vi "GetClassInfoDialog.vi"(0 "ClassWriterRefIn":refnum<class "ClassWriterNative.lvclass">, 1 "ClassItemRefIn":refnum<vi>, 5 "error in (no error)":errorcluster) -> (14 "ClassWriterRefOut":refnum<class "ClassWriterNative.lvclass">, 19 "error out":errorcluster)   [LabVIEW 2020, in "ClassWriterNative.lvclass"]
uses:
  <resource>/Framework/Providers/Open_GDS/ClassProviders/Provider_LvNativeClass/ClassWriterNative_class/ClassWriterNative.lvclass
  <resource>/Framework/Providers/Open_GDS/ClassProviders/Common/ScriptingFunctions/Scripting_ConnectorPanePatternType.ctl
  <resource>/Framework/Providers/Open_GDS/ClassProviders/Common/LvClass_class/GDSLvClass_PlugIn.ctl
  <resource>/Framework/Providers/Open_GDS/ClassProviders/Common/LvClass_class/GDSLvClass_PlugInTypes.ctl
  Instance           1 26Saved   GetClassInfoDialog .vi
  <resource>/Framework/Providers/Open_GDS/ClassProviders/Provider_LvNativeClass/ClassWriterNative_class/ClassWriterNative.lvclass/ClassWriterNative.ctl
panel:
  in  "Help":bool
  in  "_ShowContextHelp":bool
  in  "_SaveChanges":bool
  in  "_OK":bool
  out "ProductPicture":picture
  out "Connector Pane":T1 items=["4x4x4", "5x6x5", "6x8x6"]
  in  "_ClassPlugIns":T2(array[cluster]) caption="PlugIns / Design Patterns"
  in  "_EditPlugIn":bool
  out "_ClassDescription":string caption="Class description"
  out "_ClassTemplateVersion":string caption="Class Template Version"
  out "_ClassTemplateUsed":string caption="Class Template Used"
  out "_ClassProviderName":string caption="Class Provider Name"
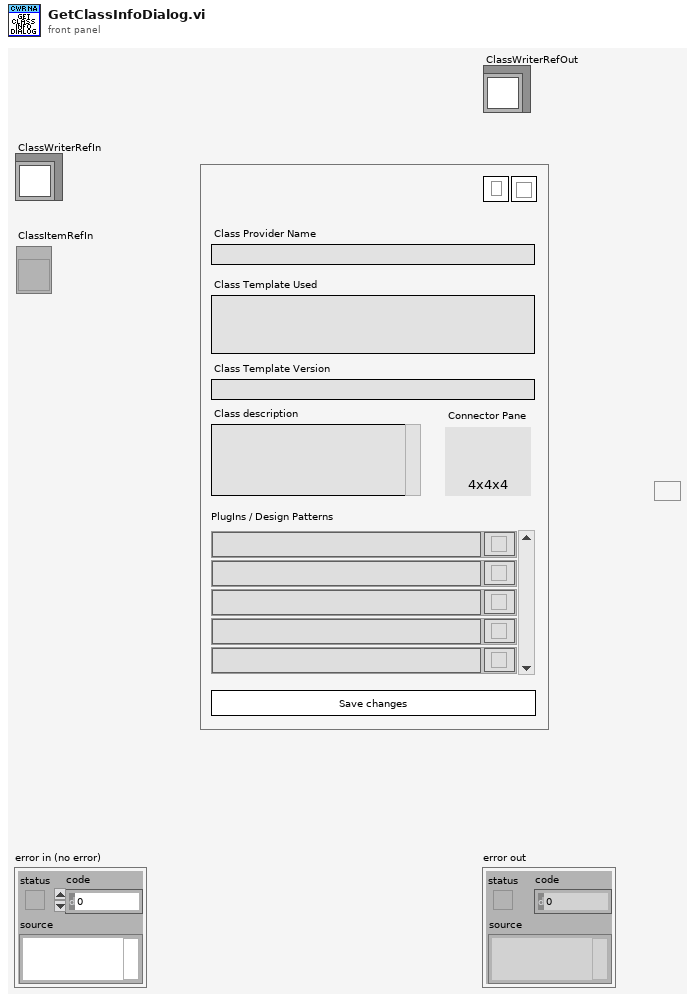
[diagram p1: front panel]
types:
  T1 = typedef "Scripting_ConnectorPanePatternType.ctl" = u16
  T2 = cluster{"_ClassPlugIn 2":string, "Remove":bool, "Block":bool}[]
  T3 = typedef "GDSLvClass_PlugIn.ctl" = cluster{"Type":T4, "ID":string, "Version":string, "Path":path, "Name":string, "Data":variant}
  T4 = typedef "GDSLvClass_PlugInTypes.ctl" = enum16{"DesignPattern", "MethodTypes"}
  T5 = cluster{"_ClassPlugIn 2":string, "_RemovePlugIn":bool, "Block":bool}
  T6 = typedef "GDSLvCLass_ClassSettingsType.ctl" = cluster{"ClassProviderName":string, "ClassTemplateUsed":string, "ClassTemplateVersion":string, "ClassDescription":string, "PlugIns":T3[], "ConnectorPanePattern":string}
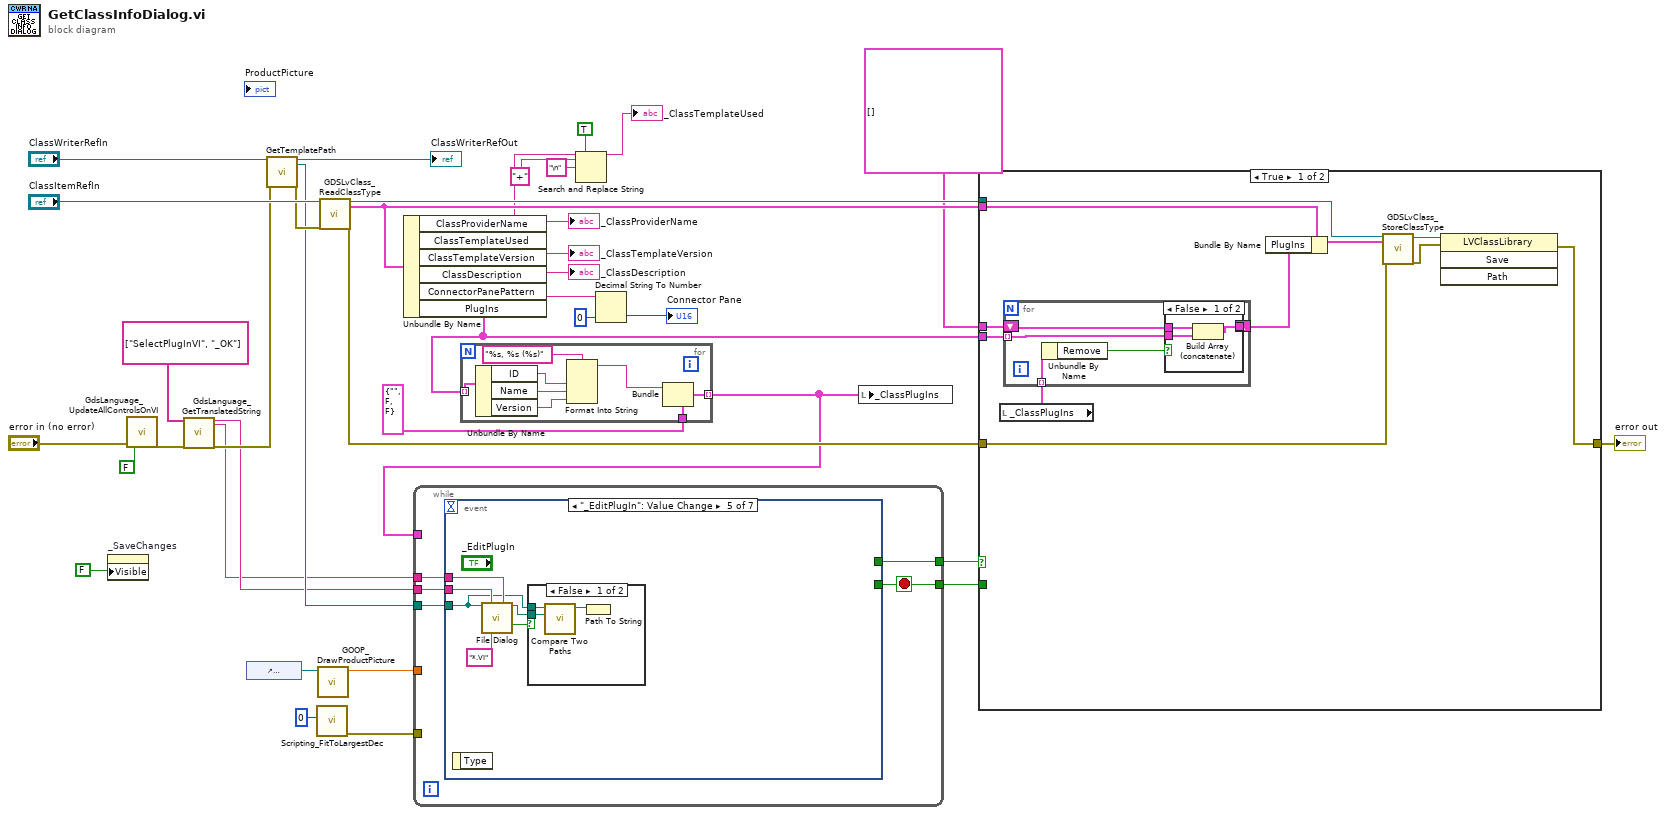
[diagram p0: block diagram]
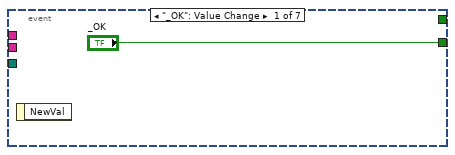
[diagram p4: hidden frame]
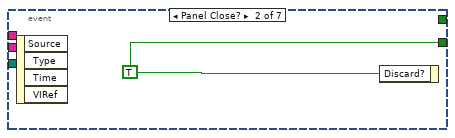
[diagram p5: hidden frame]
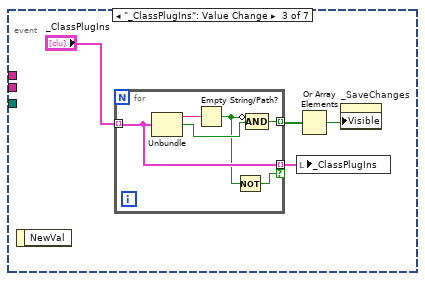
[diagram p6: hidden frame]
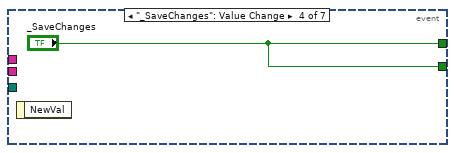
[diagram p7: hidden frame]
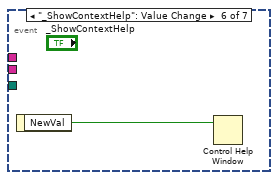
[diagram p9: hidden frame]
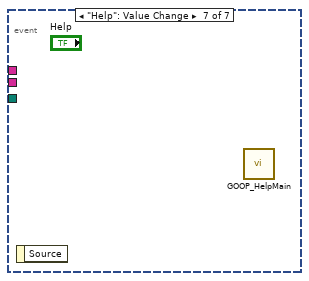
[diagram p10: hidden frame]
diagram:
  n1 = property on="_SaveChanges" class="Bool"("Visible"=FALSE) -> ()  [unwired: 2 in, 2 out]
  n2 = call <resource>:"GdsLanguage_UpdateAllControlsOnVI.vi"("error in (no error)"="error in (no error)", "CreateLanguageFile(Use this to create a languageFile)"=FALSE) -> ("error out"=w24:errorcluster)  [unwired: 16 in, 1 out]
  n3 = call <resource>:"GdsLanguage_GetTranslatedString.vi"("StringID(s)"=string[] ["SelectPlugInVI", "_OK"], "error in (no error)"=w24) -> ("FirstStringOut"=w21:string, "SecondStringOut"=w19:string, "error out"=w23:errorcluster)  [unwired: 14 in, 1 out]
  n4 = control-ref of="ProductPicture"() -> (w4:refnum<vi>)
  n5 = call-dynamic "GetTemplatePath.vi"("reference in"="ClassWriterRefIn", "error in (no error)"=w23) -> ("reference out"=→"ClassWriterRefOut":refnum<class "ClassWriterNative.lvclass">, "FolderPathOut"=w22:path, "error out"=w26:errorcluster)  [unwired: 13 in, 2 out]
  n6 = call <resource>:"Scripting_FitToLargestDec.vi"("border spacing (2 px)"=0) -> ("error out"=w1:errorcluster)  [unwired: 5 in, 1 out]
  n7 = call <resource>:"GOOP_DrawProductPicture.vi"("ProductPictureControl"=w4) -> ("Zoom Factor"=w3:sgl)  [unwired: 10 in]
  n8 = call <resource>:"GDSLvClass_ReadClassType.vi"("Class Refnum In"="ClassItemRefIn", "error in (no error)"=w26) -> ("Class Refnum Out"=w34:refnum<vi>, "ClassSettings"=w29:T6, "error out"=w33:errorcluster)  [unwired: 15 in]
  n9 = Unbundle By Name(w29) -> ("ClassProviderName"=→"_ClassProviderName":string, "ClassTemplateUsed"=w13:string, "ClassTemplateVersion"=→"_ClassTemplateVersion":string, "ClassDescription"=→"_ClassDescription":string, "ConnectorPanePattern"=w8:string, "PlugIns"=w16:T3[])
  n10 = for {
    tunnel: w16 -> [w44] mode=indexing
    tunnel: T5 {"_ClassPlugIn 2"="", "_RemovePlugIn"=FALSE, "Block"=FALSE} ("Cluster") -> [w46]
    tunnel: [w45] -> w5 mode=indexing
    n11 = Unbundle By Name(w44) -> ("ID"=w41:string, "Name"=w40:string, "Version"=w39:string)
    n12 = Format Into String(format string="%s, %s (%s)", w41, w40, w39) -> (resulting string=w42:string)  [unwired: 2 in, 1 out]
    n13 = Bundle(cluster=w46, "_ClassPlugIn 2"=w42) -> (w45:T5)  [unwired: 2 in]
  }
  n14 = while {
    tunnel: [w51] -> w28
    tunnel: w22 -> [w50]
    tunnel: w21 -> [w49]
    tunnel: w19 -> [w48]
    tunnel: [w47] -> w14
    tunnel: w5 -> [_]
    tunnel: w3 -> [_]
    tunnel: w1 -> [_]
    stop <- w51 stop-if-true
    n15 = event shown="[4] \"_EditPlugIn\": Value Change" {
      selector: _ -> [_ _ _ _ _ _ _]
      dyn-events: _ -> [_ _ _ _ _ _ _]
      timeout: _ -> [_ _ _ _ _ _ _]
      tunnel: ["_OK" w53 _ "_SaveChanges" _ _ _] -> w51
      tunnel: w50 -> [_ _ _ _ w66 _ _]
      tunnel: w49 -> [_ _ _ _ w70 _ _]
      tunnel: w48 -> [_ _ _ _ w68 _ _]
      tunnel: [_ _ _ "_SaveChanges" _ _ _] -> w47
      event "_OK": Value Change {
        n16 = event-data() -> ()  [unwired: 1 in, 1 out]
      }
      event Panel Close? {
        w53 = TRUE ("Discard?")
        n17 = event-data() -> ()  [unwired: 1 in, 4 out]
        n18 = event-data("Discard?"=w53) -> ()  [unwired: 1 in, 1 out]
      }
      event "_ClassPlugIns": Value Change {
        n19 = event-data() -> ()  [unwired: 1 in, 1 out]
        n20 = for {
          tunnel: "_ClassPlugIns" -> [w61] mode=indexing
          tunnel: [w61] -> w56 mode=indexing if=w59
          tunnel: [w58] -> w55 mode=indexing
          n21 = Unbundle(w61) -> ("_ClassPlugIn 2"=w63:string, "Remove"=w62:bool)  [unwired: 1 out]
          n22 = Empty String/Path?(string/path=w63) -> (empty?=w60:bool)
          n23 = Not(x=w60) -> (.not. x?=w59:bool)
          n24 = Compound Arithmetic op=AND(invert w60, w62) -> (w58:bool)
        }
        n25 = local write "_ClassPlugIns"(w56) -> ()
        n26 = Or Array Elements(Boolean array=w55) -> (logical OR=w54:bool)
        n27 = property on="_SaveChanges" class="Bool"("Visible"=w54) -> ()  [unwired: 2 in, 2 out]
      }
      event "_SaveChanges": Value Change {
        n28 = event-data() -> ()  [unwired: 1 in, 1 out]
      }
      event "_EditPlugIn": Value Change {
        n29 = event-data() -> ()  [unwired: 1 in, 1 out]
        n30 = call "File Dialog"("start path"=w66, "prompt"=w70, "button label"=w68, "pattern (all files)"="*.VI") -> ("selected path"=w65:path, "cancelled"=w67:bool)  [unwired: 8 in, 2 out]
        n31 = case shown="False" w67 {
          tunnel: w66 -> [w73 _]
          tunnel: w65 -> [w72 _]
          frame False {
            n32 = call <vilib>:"Compare Two Paths.vi"("Path 2"=w72, "Path 1"=w73) -> ("Relative Path from 1 to 2"=w71:path)  [unwired: 6 in, 3 out]
            n33 = Path To String(path=w71) -> ()  [unwired: 1 out]
          }
          frame True {
          }
        }
      }
      event "_ShowContextHelp": Value Change {
        n34 = event-data() -> ("NewVal"=w74:bool)  [unwired: 1 in]
        n35 = Control Help Window(1:w74) -> ()  [unwired: 1 in]
      }
      event "Help": Value Change {
        n36 = event-data() -> ()  [unwired: 1 in, 1 out]
        n37 = call <resource>:"GOOP_HelpMain.vi"() -> ()  [unwired: 12 in]
      }
    }
  }
  n38 = Search and Replace String(replace all?=TRUE ("replace all? (F)"), input string=w13, search string="+", replace string="\n" ("replace string (\"\")")) -> (result string=→"_ClassTemplateUsed":string)  [unwired: 4 in, 3 out]
  n39 = Decimal String To Number(string=w8, default (0L)=u16 0 ("default (0 I32)")) -> (number=→"Connector Pane":u16)  [unwired: 1 in, 1 out]
  n40 = local write "_ClassPlugIns"(w5) -> ()
  n41 = case shown="True" w14 {
    tunnel: w34 -> [w85 _]
    tunnel: w33 -> [w84 w95]
    tunnel: [w83 w95] -> w32
    tunnel: w29 -> [w82 _]
    tunnel: w28 -> [_ _]
    tunnel: w16 -> [w80 _]
    tunnel: T3[] [] -> [w78 _]
    frame True {
      n42 = local read "_ClassPlugIns"() -> (w77:T2)
      n43 = for {
        tunnel: w80 -> [w88] mode=indexing
        shift-right: [w89] -> w79
        shift-left: w78 -> [w90]
        tunnel: w77 -> [w87] mode=indexing
        n44 = Unbundle By Name(w87) -> ("Remove"=w86:bool)
        n45 = case shown="False" w86 {
          tunnel: w90 -> [w93 w94]
          tunnel: w88 -> [w92 _]
          tunnel: [w91 w94] -> w89
          frame False {
            n46 = Build Array (concatenate)(w93, w92) -> (w91:T3[])
          }
          frame True {
          }
        }
      }
      n47 = Bundle By Name(cluster=w82, "PlugIns"=w79) -> (w81:T6)
      n48 = call <resource>:"GDSLvClass_StoreClassType.vi"("Class Refnum In"=w85, "ClassSettings"=w81, "error in (no error)"=w84) -> ("Class Refnum Out"=w76:refnum<vi>, "error out"=w75:errorcluster)  [unwired: 15 in]
      n49 = invoke class="LVClassLibrary" method="Save"(reference=w76, error in=w75) -> (error out=w83:errorcluster)  [unwired: 2 in, 3 out]
    }
    frame False {
    }
  }
  "error out" <- w32
